vi "set Frequency Line.vi"(8 "error in (no error)":errorcluster, 10 "Frequency Line (Hz)":T1 {"Line 2" format="%#_6p"; "Line 1" format="%#_6p"}, 11 "FSV-40N in":refnum<class "FSV-40N.lvclass">) -> (0 "error out":errorcluster, 3 "FSV-40N out":refnum<class "FSV-40N.lvclass">)   [LabVIEW 2023, in "Spectrum Analyzer.lvlib" / "FSV-40N.lvclass"]
uses:
  FSV-40N.lvclass
  TYPE DEFINITION/TYPE Frequency Line Param.ctl
  FSV-40N.lvclass/FSV-40N.ctl
  Spectrum Analyzer.lvlib
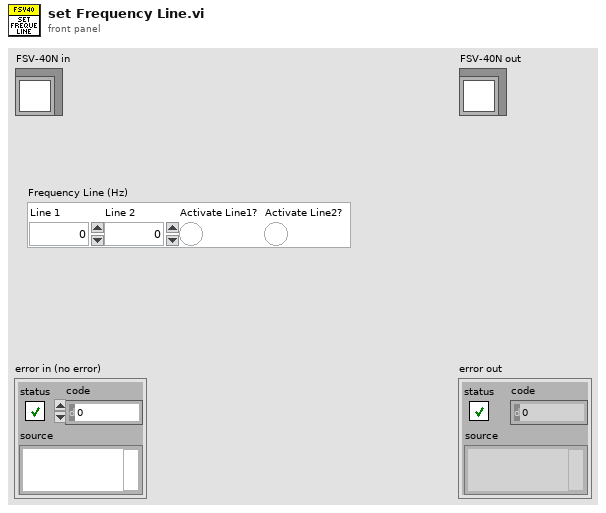
[diagram p1: front panel]
types:
  T1 = typedef "Spectrum Analyzer.lvlib/TYPE Frequency Line Param.ctl" = cluster{"Line 1":dbl, "Line 2":dbl, "Activate Line1?":bool, "Activate Line2?":bool}
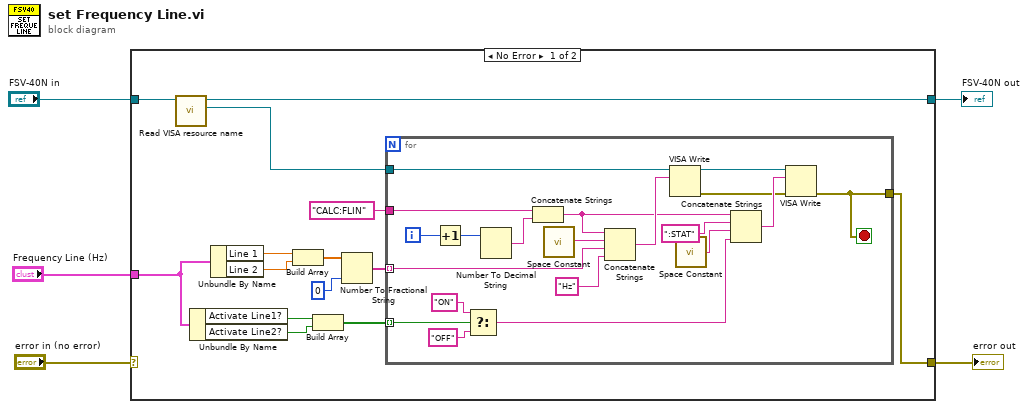
[diagram p0: block diagram]
diagram:
  n1 = case shown="No Error" "error in (no error)" {
    selector: "error in (no error)" -> [_ w40]
    tunnel: "FSV-40N in" -> [w19 w41]
    tunnel: [w6 w41] -> w4
    tunnel: [w7 w40] -> w2
    tunnel: "Frequency Line (Hz)" -> [w11 _]
    frame No Error {
      n2 = call "Read VISA resource name.vi"("FSV-40N in"=w19) -> ("VISA resource name"=w18:refnum<visa-resource-name>, "FSV-40N out"=w6:refnum<class "FSV-40N.lvclass">)  [unwired: 8 in, 1 out]
      n3 = Unbundle By Name(w11) -> ("Activate Line1?"=w10:bool, "Activate Line2?"=w9:bool)
      n4 = Unbundle By Name(w11) -> ("Line 1"=w17:dbl, "Line 2"=w16:dbl)
      n5 = Build Array(w17, w16) -> (w15:dbl[])
      n6 = Build Array(w10, w9) -> (w8:bool[])
      n7 = Number To Fractional String(number=w15, precision (6)=i16 0) -> (F-format string=w13:string[])  [unwired: 2 in]
      n8 = for {
        tunnel: w18 -> [w39]
        tunnel: w13 -> [w32] mode=indexing
        tunnel: "CALC:FLIN" ("write buffer") -> [w35]
        tunnel: w8 -> [w26] mode=indexing
        tunnel: [w20] -> w7
        i -> [w37]
        stop <- w20 stop-if-true
        n9 = Increment(x=w37) -> (x+1=w36:i32)
        n10 = Select(t="ON" ("string"), s=w26, f="OFF") -> (s? t:f=w23:string)
        n11 = Number To Decimal String(number=w36) -> (decimal integer string=w34:string)  [unwired: 1 in]
        n12 = Concatenate Strings(w35, w34) -> (w29:string)
        n13 = call <vilib>:"Space Constant.vi"() -> ("String"=w33:string)
        n14 = Concatenate Strings(w29, w33, w32, "Hz" ("string")) -> (w30:string)
        n15 = VISA Write(VISA resource name=w39, write buffer=w30) -> (VISA resource name out=w38:refnum<visa-resource-name>, error out=w21:errorcluster)  [unwired: 1 in, 1 out]
        n16 = call <vilib>:"Space Constant.vi"() -> ("String"=w27:string)
        n17 = Concatenate Strings(w29, ":STAT" ("string"), w27, w23) -> (w22:string)
        n18 = VISA Write(VISA resource name=w38, write buffer=w22, error in (no error)=w21) -> (error out=w20:errorcluster)  [unwired: 2 out]
      }
    }
    frame Error {
    }
  }
  "error out" <- w2
  "FSV-40N out" <- w4
